vi "Wait for Turn Table Movement Complete.vi"(8 "error in (no error)":errorcluster, 11 "AUDIX EM1000 in":refnum<class "AUDIX EM1000.lvclass">) -> (0 "error out":errorcluster, 3 "AUDIX EM1000 out":refnum<class "AUDIX EM1000.lvclass">)   [LabVIEW 2023, in "Turn Table and Mast.lvlib" / "AUDIX EM1000.lvclass"]
uses:
  AUDIX EM1000.lvclass
  AUDIX EM1000.lvclass/AUDIX EM1000.ctl
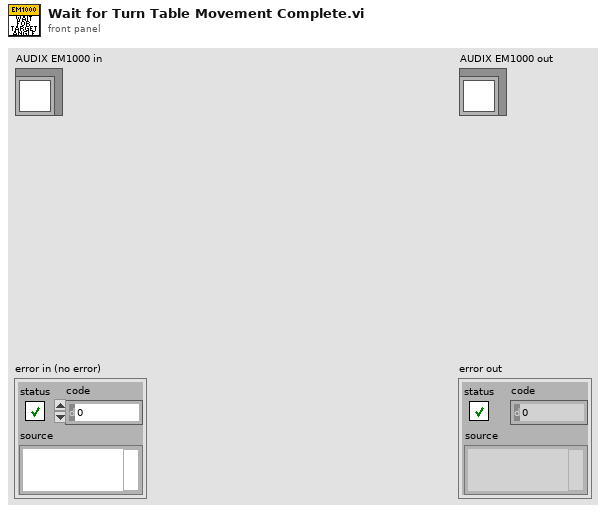
[diagram p1: front panel]
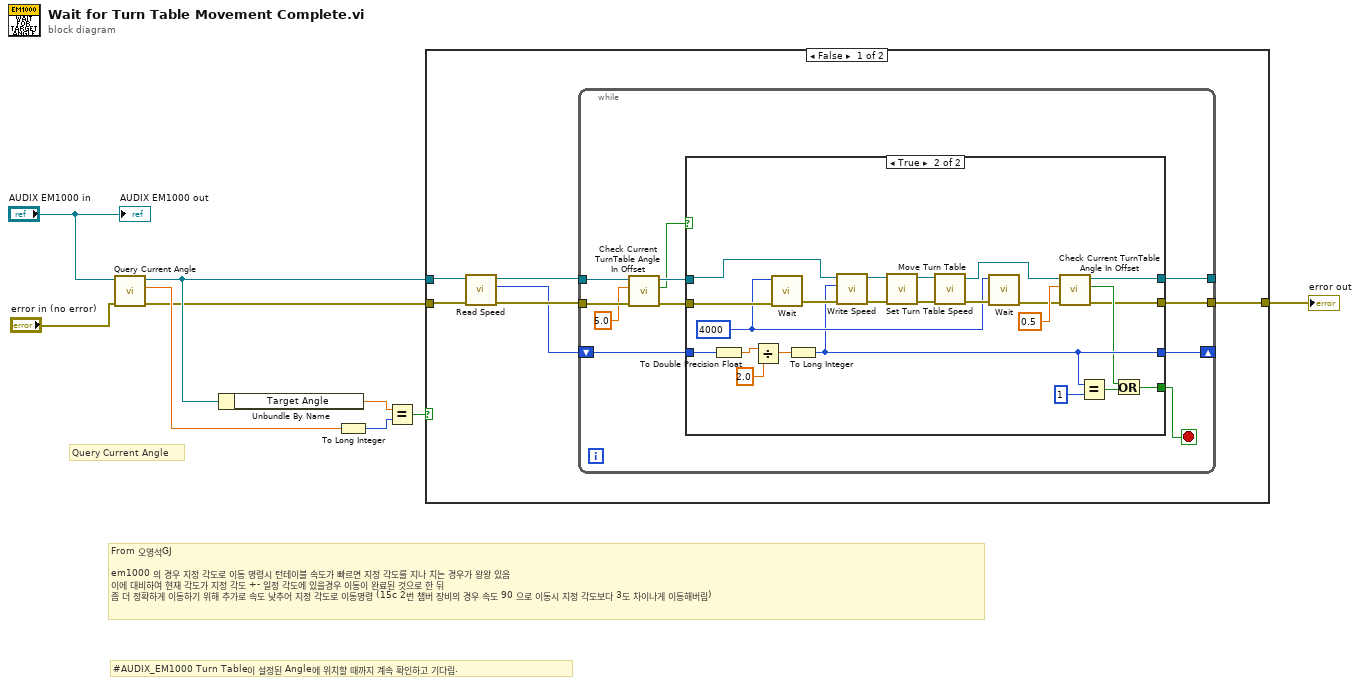
[diagram p0: block diagram]
diagram:
  # "From 오영석GJ\n\nem1000 의 경우 지정 각도로 이동 명령시 턴테이블 속도가 빠르면 지정 각도를 지나 치는 경우가 왕왕 있음\n이에 대비하여 현재 각도가 지정 각도 +- 일정 각도에 있을경우 이동이 완료된 것으로 한 뒤\n좀 더 정확하게 이동하기 위해 추가로 속도 낮추어 지정 각도로 이동명령 (15c 2번 챔버 장비의 경우 속도 90 으로 이동시 지정 각도보다 3도 차이나게 이동해버림)"
  # "Query Current Angle"
  # "#AUDIX_EM1000 Turn Table이 설정된 Angle에 위치할 때까지 계속 확인하고 기다림."
  n1 = call-dynamic "Query Current Angle.vi"("error in (no error)"="error in (no error)", "AUDIX EM1000 in"="AUDIX EM1000 in") -> ("error out"=w3:errorcluster, "Current Angle"=w8:dbl, "AUDIX EM1000 out"=w4:refnum<class "AUDIX EM1000.lvclass">)  [unwired: 7 in]
  n2 = Unbundle By Name(w4) -> ("Target Angle"=w7:dbl)
  n3 = To Long Integer(number=w8) -> (32bit integer=w6:i32)
  n4 = Equal?(x=w7, y=w6) -> (x = y?=w5:bool)
  n5 = case shown="False" w5 {
    tunnel: w4 -> [w15 _]
    tunnel: w3 -> [w14 w53]
    tunnel: [w10 w53] -> w2
    frame False {
      n6 = call "Read Speed.vi"("error in (no error)"=w14, "AUDIX EM1000 in"=w15) -> ("error out"=w12:errorcluster, "Speed"=w11:i32, "AUDIX EM1000 out"=w13:refnum<class "AUDIX EM1000.lvclass">)  [unwired: 7 in]
      n7 = while {
        tunnel: w13 -> [w23]
        tunnel: w12 -> [w24]
        shift-right: [w25] -> _
        shift-left: w11 -> [w26]
        tunnel: [w17] -> _
        tunnel: [w16] -> w10
        stop <- w18 stop-if-true
        n8 = call-dynamic "Check Current TurnTable Angle In Offset.vi"("error in (no error)"=w24, "Current Angle"=5.0 ("Target Offset"), "AUDIX EM1000 in"=w23) -> ("error out"=w20:errorcluster, "In Offset Range?"=w19:bool, "AUDIX EM1000 out"=w21:refnum<class "AUDIX EM1000.lvclass">)  [unwired: 6 in]
        n9 = case shown="True" w19 {
          tunnel: w21 -> [w28 w47]
          tunnel: w20 -> [w27 w52]
          tunnel: w26 -> [w29 w51]
          tunnel: [w29 w36] -> w25
          tunnel: [_ w32] -> w18
          tunnel: [w28 w31] -> w17
          tunnel: [w27 w30] -> w16
          frame False {
          }
          frame True {
            w39 = u32 4000 ("대기 시간 (ms)")
            n10 = To Double Precision Float(number=w51) -> (double precision float=w50:dbl)
            n11 = Divide(x=w50, y=2.0) -> (x/y=w46:dbl)
            n12 = call "Wait.vi"("에러 상수 입력"=w52, "대기 시간 (ms)"=w39) -> ("에러 상수 출력"=w48:errorcluster)  [unwired: 9 in]
            n13 = To Long Integer(number=w46) -> (32bit integer=w36:i32)
            n14 = call "Write Speed.vi"("error in (no error)"=w48, "Speed"=w36, "AUDIX EM1000 in"=w47) -> ("error out"=w44:errorcluster, "AUDIX EM1000 out"=w45:refnum<class "AUDIX EM1000.lvclass">)  [unwired: 7 in]
            n15 = call-dynamic "Set Turn Table Speed.vi"("error in (no error)"=w44, "AUDIX EM1000 in"=w45) -> ("error out"=w42:errorcluster, "AUDIX EM1000 out"=w43:refnum<class "AUDIX EM1000.lvclass">)  [unwired: 8 in]
            n16 = call-dynamic "Move Turn Table.vi"("error in (no error)"=w42, "AUDIX EM1000 in"=w43) -> ("error out"=w40:errorcluster, "AUDIX EM1000 out"=w37:refnum<class "AUDIX EM1000.lvclass">)  [unwired: 8 in]
            n17 = call "Wait.vi"("에러 상수 입력"=w40, "대기 시간 (ms)"=w39) -> ("에러 상수 출력"=w38:errorcluster)  [unwired: 9 in]
            n18 = call-dynamic "Check Current TurnTable Angle In Offset.vi"("error in (no error)"=w38, "Current Angle"=0.5 ("Target Offset"), "AUDIX EM1000 in"=w37) -> ("error out"=w30:errorcluster, "In Offset Range?"=w33:bool, "AUDIX EM1000 out"=w31:refnum<class "AUDIX EM1000.lvclass">)  [unwired: 6 in]
            n19 = Equal?(x=w36, y=1) -> (x = y?=w34:bool)
            n20 = Or(x=w33, y=w34) -> (x .or. y?=w32:bool)
          }
        }
      }
    }
    frame True {
    }
  }
  "error out" <- w2
  "AUDIX EM1000 out" <- "AUDIX EM1000 in"
